vi "Set TestData.vi"(8 "error in (no error)":errorcluster, 9 "Main":refnum<vi>, 10 "Test Index":i32, 11 "3way Lap In":refnum<class "3way Lap.lvclass">) -> (0 "error out":errorcluster, 2 "Test Data":cluster{"Best Linear Fit":dbl[], "Y":dbl[]}[](array[cluster]), 3 "3way Lap  out":refnum<class "3way Lap.lvclass">)   [LabVIEW 2025, in "Flow Grind.lvlib" / "3way Lap.lvclass"]
uses:
  3way Lap.lvclass
  3way Lap.lvclass/3way Lap.ctl
  <vilib>/Analysis/6fits.llb/Curve Fitting Criteria.ctl
  1fd75abc-c2ef-4fe7-a3c8-a47552fa74cb.vi
  <vilib>/Array/Sort 2D Array - Pop Stack.vi
  <vilib>/Array/Sort 2D Array - Push Stack.vi
  1fd75abc-c2ef-4fe7-a3c8-a47552fa74cb.vi/269d4b3b-47f5-49e3-8884-44851e4dd9d5.vi
  1fd75abc-c2ef-4fe7-a3c8-a47552fa74cb.vi/6d99389c-673d-4efb-bf33-19b32bcf4cf8.vi
  <vilib>/Analysis/NI_AALPro.lvlib
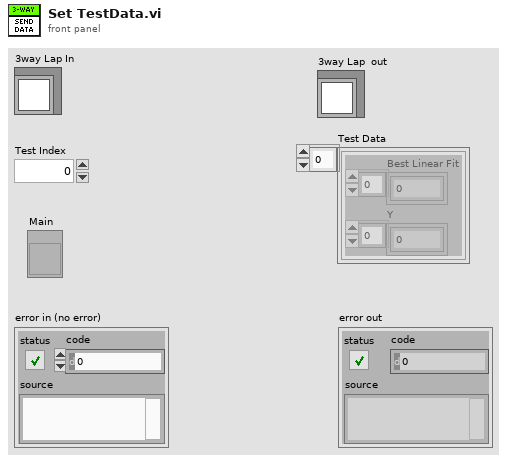
[diagram p1: front panel]
types:
  T1 = typedef "NI_AALPro.lvlib/Curve Fitting Criteria.ctl" = u16
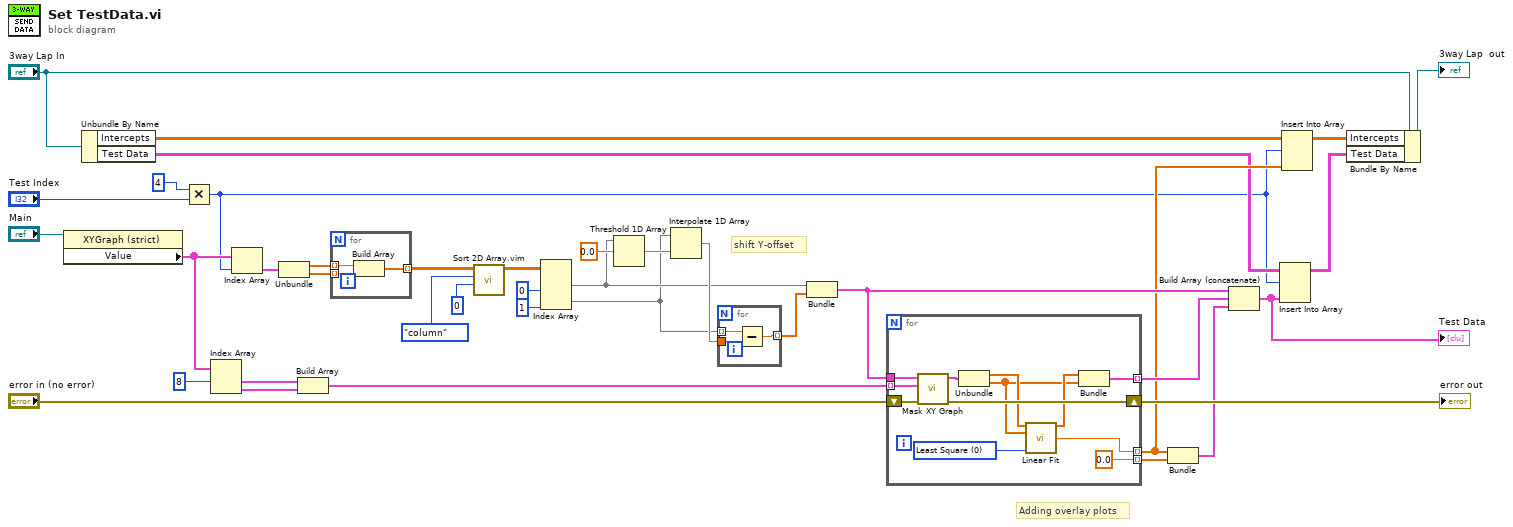
[diagram p0: block diagram]
diagram:
  # "Adding overlay plots"
  # "shift Y-offset"
  n1 = property class="XYGraph (strict)"(reference="Main") -> ("Value"=w9:cluster{dbl[], dbl[]}[])  [unwired: 1 in, 2 out]
  n2 = Unbundle By Name("3way Lap In") -> ("Intercepts"=w15:dbl[][], "Test Data"=w12:cluster{"Best Linear Fit":dbl[], "Y":dbl[]}[][])
  n3 = Multiply(x=4, y="Test Index") -> (x*y=w1:i32)
  n4 = Index Array(array=w9, index #1=8 ("index")) -> (element #1=w7:cluster{dbl[], dbl[]}, element #2=w6:cluster{dbl[], dbl[]})  [unwired: 1 in]
  n5 = Index Array(array=w9, index=w1) -> (element=w19:cluster{dbl[], dbl[]})
  n6 = Unbundle(w19) -> (w18:dbl[], w32:dbl[])
  n7 = Build Array(w7, w6) -> (w5:cluster{dbl[], dbl[]}[])
  n8 = for {
    tunnel: w18 -> [w41] mode=indexing
    tunnel: w32 -> [w40] mode=indexing
    tunnel: [w39] -> w33 mode=indexing
    n9 = Build Array(w41, w40) -> (w39:dbl[])
  }
  n10 = call "Sort 2D Array.vim"("index"=0, "dimension to index (column)"=enum16{"column", "row"}."column", "2D array"=w33) -> ("sorted 2D array"=w36:dbl[][])  [unwired: 7 in, 1 out]
  n11 = Index Array(array=w36, index (col) #1=0 ("index (row)"), index (col) #2=1 ("index (col)")) -> (element #1=w27:dbl[], element #2=w26:dbl[])  [unwired: 2 in]
  n12 = Threshold 1D Array(2:0.0 ("fractional index or x"), 3:w27) -> (0:w29:dbl)  [unwired: 1 in]
  n13 = Interpolate 1D Array(1:w29, 2:w26) -> (0:w38:dbl)
  n14 = for {
    tunnel: w38 -> [w43]
    tunnel: [w44] -> w28 mode=indexing
    tunnel: w26 -> [w42] mode=indexing
    n15 = Subtract(x=w42, y=w43) -> (x-y=w44:dbl)
  }
  n16 = Bundle("sorted 2D array"=w27, w28) -> (w21:cluster{"sorted 2D array":dbl[], dbl[]})  [unwired: 1 in]
  n17 = for {
    tunnel: w21 -> [w56]
    tunnel: w5 -> [w55] mode=indexing
    shift-right: [w53] -> w24
    shift-left: "error in (no error)" -> [w54]
    tunnel: [w51] -> w23 mode=indexing
    tunnel: [w45] -> w14 mode=indexing
    tunnel: [0.0 ("fractional index or x")] -> w20 mode=indexing
    w49 = T1 0 items=["Least Square", "Least Absolute Residual", "Bisquare"] ("method")
    n18 = call "Mask XY Graph.vi"("error in (no error)"=w54, "Mask"=w55, "Data"=w56) -> ("error out"=w53:errorcluster, "Masked Data"=w52:cluster{"X":dbl[], "Y":dbl[]})  [unwired: 6 in, 1 out]
    n19 = Unbundle(w52) -> ("X"=w48:dbl[], "Y"=w46:dbl[])
    n20 = call <vilib>:"Linear Fit.vi"("Y"=w48, "X"=w46, "method"=w49) -> ("Best Linear Fit"=w47:dbl[], "intercept"=w45:dbl)  [unwired: 8 in, 3 out]
    n21 = Bundle("Best Linear Fit"=w47, "Y"=w46) -> (w51:cluster{"Best Linear Fit":dbl[], "Y":dbl[]})  [unwired: 1 in]
  }
  "error out" <- w24
  n22 = Bundle(w14, w20) -> (w22:cluster{dbl[], dbl[]})  [unwired: 1 in]
  n23 = Build Array (concatenate)(w21, w23, w22) -> (w4:cluster{"Best Linear Fit":dbl[], "Y":dbl[]}[])
  "Test Data" <- w4
  n24 = Insert Into Array(array=w12, index (row)=w1, new element=w4) -> (w11:cluster{"Best Linear Fit":dbl[], "Y":dbl[]}[][])  [unwired: 1 in]
  n25 = Insert Into Array(array=w15, index (row)=w1, new element=w14) -> (w13:dbl[][])  [unwired: 1 in]
  n26 = Bundle By Name(cluster="3way Lap In", "Intercepts"=w13, "Test Data"=w11) -> (→"3way Lap  out":refnum<class "3way Lap.lvclass">)
